vi "MongoDB.Database.AddUser.vi"(8 "error in (no error)":errorcluster, 10 "Username":string, 11 "MongoDB.Database in":refnum<class "MongoDB.Database.lvclass">) -> (0 "error out":errorcluster, 3 "MongoDB.Database out":refnum<class "MongoDB.Database.lvclass">)   [LabVIEW 2014, in "MongoDB.Database.lvclass"]
uses:
  MongoDB.Database.lvclass
  C:/Users/Richard/Documents/GitHub/mongo-labview-driver/CSharp/bin/MongoDB.Driver.Legacy.dll
  CSharp/bin/MongoDB.Driver.Legacy.dll
  MongoDB.Database.lvclass/MongoDB.Database.ctl
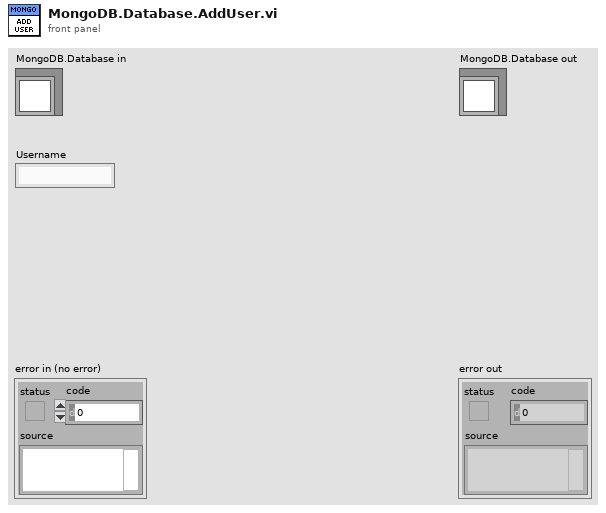
[diagram p1: front panel]
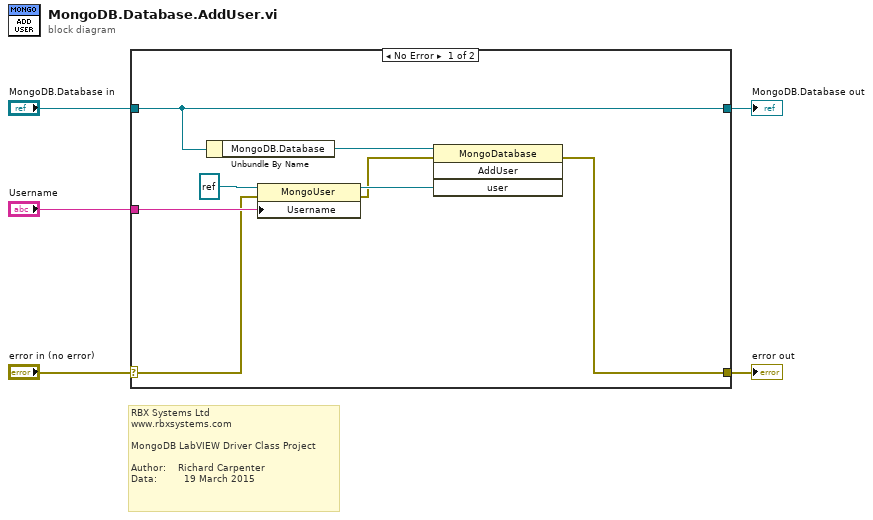
[diagram p0: block diagram]
diagram:
  # "RBX Systems Ltd\nwww.rbxsystems.com\n\nMongoDB LabVIEW Driver Class Project\n\nAuthor:    Richard Carpenter\nData:         19 March 2015"
  n1 = case shown="No Error" "error in (no error)" {
    selector: "error in (no error)" -> [w6 w15]
    tunnel: [w7 w15] -> w4
    tunnel: [w13 w14] -> w2
    tunnel: "MongoDB.Database in" -> [w13 w14]
    tunnel: "Username" -> [w9 _]
    frame No Error {
      n2 = Unbundle By Name(w13) -> ("MongoDB.Database"=w12:refnum<k24>)
      n3 = property class="MongoUser"(reference=refnum<k24> refnum ("user"), error in=w6, "Username"=w9) -> (reference out=w10:refnum<k24>, error out=w8:errorcluster)
      n4 = invoke class="MongoDatabase" method="AddUser"(reference=w12, error in=w8, "user"=w10) -> (error out=w7:errorcluster)  [unwired: 1 in, 3 out]
    }
    frame Error {
    }
  }
  "error out" <- w4
  "MongoDB.Database out" <- w2
